vi "APU Synchronization Trigger.vi"(6 "trigger line.<user name>":refnum<k21>="PXI_Trig0", 11 "send trigger.<user name>":bool) -> ()   [LabVIEW 2015, in "Engine Simulation Toolkit.lvlib" / "APU.lvlib"]
doc: "Sends triggers on <b>trigger line.<user name></b> to keep multiple FPGAs running a single APU synchronized.\n\n<b>trigger line.<user name></b> - the PXI trigger line to use for FPGA synchronization. Connect this same trigger line value to the trigger line linput of <b>Create APU Register Bus - Multi FPGA.vi</b>.\n<b>send trigger.<user name></b> - sends a trigger on the trigger line across the PXI backplane. Create a control for this and make sure the mechanical action is set to <b>Latch When Released</b>."
uses:
  APU.lvlib
  <vilib>/rvi/eio/common/nirviEmuTemplateMethod_errors.vi
  <vilib>/eio/EIOMethodNode/EIOMethodNode.xnode
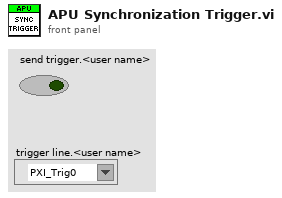
[diagram p1: front panel]
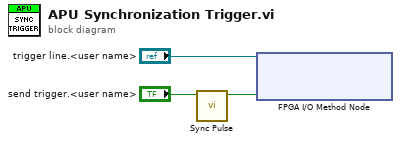
[diagram p0: block diagram]
diagram:
  n1 = call "Sync Pulse.vi"("Sync"="send trigger.<user name>") -> ("Sync Enable?"=w1:bool)  [unwired: 10 in]
  n2 = xnode "FPGA I/O Method Node"("FPGA I/O In"="trigger line.<user name>", "Enable"=w1) -> ()  [unwired: 1 out]
